vi "RT Driver VI.vi"(7 "Operation":T1, 11 "Device Reference in":T2 format="%.0x") -> (0 "Error Code":i32)   [LabVIEW 2020, in "FPGA Addon Engine.lvlib"]
uses:
  FPGA Addon Engine.lvlib
  <vilib>/rvi/interface/nirviCloseFPGA/nirviCloseFPGA.xnode
  <vilib>/NI VeriStand/Custom Device API/Custom Device API.lvlib
  Processes/Input DMA Engine.vi
  <vilib>/rvi/interface/nirviMethod/nirviMethod.xnode
  Processes/Output DMA Engine.vi
  <vilib>/NI/NIVS Inline Async API/_VS Inline Async API/VS Inline Async API/VS Inline Async API.lvclass
  <vilib>/NI/NIVS Inline Async API/_VS Inline Async API/VS Inline Async API/Types/Error Handling Settings.ctl
  <vilib>/rvi/interface/nirviMethod/StockFPGA_InlinedMethodWaitForSingleIRQ.vi
  <vilib>/FPGAPlugInAG/Dynamic/niLvFpga_WaitOnIrq_Dynamic.vi
  <vilib>/FPGAPlugInAG/Dynamic/niLvFpga_AcknowledgeIrq_Dynamic.vi
  <vilib>/FPGAPlugInAG/Dynamic/niLvFpga_Close_Dynamic.vi
  <vilib>/NI VeriStand/Custom Device Waveform API/Multiple Waveforms Write (DBL)/Multiple Waveforms Write (DBL).lvclass
  <vilib>/NI VeriStand/Custom Device Waveform API/Single Waveform Read (DBL)/Single Waveform Read (DBL).lvclass
  <vilib>/NI VeriStand/Custom Device API/Custom Device Item Ref.ctl
  <vilib>/NI VeriStand/Custom Device API/Hardware Interface Driver VI Operation.ctl
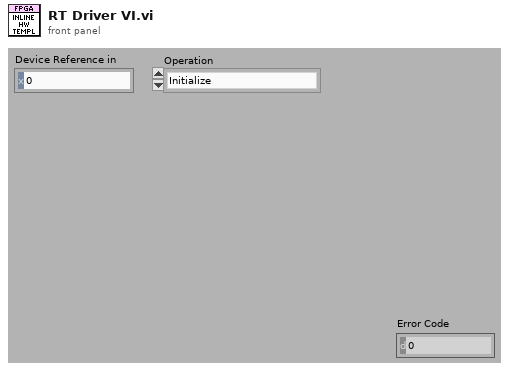
[diagram p1: front panel]
types:
  T1 = typedef "Custom Device API.lvlib/Hardware Interface Driver VI Operation.ctl" = enum16{"Initialize", "Start", "Read Data from HW", "Write Data to HW", "Close"}
  T2 = typedef "Custom Device API.lvlib/Custom Device Item Ref.ctl" = u64
  T3 = typedef "FPGA Addon Engine.lvlib/State Variables.ctl" = cluster{"FPGA Ref":refnum<k20>, "IncomingRegisters.Refs":T4[], "IncomingDMA.Refs":T7[], "OutgoingRegisters.Refs":T4[], "OutgoingDMA.Refs":T12[], "Compiled":T14}
  T4 = typedef "FPGA Addon Engine.lvlib/Register Settings.ctl" = cluster{"Name":string, "Data Type":T5, "session":u32, "Scalar Type":T6, "Index":i32, "Length":i32, "attributes":variant, "default value":variant, "RegisterOffset":u32}
  T5 = typedef "FPGA Addon Shared.lvlib/FPGA Addon Data Type.ctl" = enum8{"<Null>", "I8", "I16", "I32", "I64", "U8", "U16", "U32", "U64", "SGL", "Boolean", "Analog PWM In Settings", "Analog PWM In", "Digital PWM In Settings", "Digital PWM In", "Digital PWM Out", "Sine Out", "FXP", "FXP+/-24.5", "FXP+/-16.5", "FXP+/-32.8", "FXP+/-64.32", "FXP+/-16.7", "FXP+/-20.5", "FXP+/-27.5", "FXP+/-32.16", "FXP+16.3", "FXP+18.3", "Digital Static In", "Digital Static Out", "Digital Static In Settings", "Digital WSS Out", "Quad Encoder Settings", "Quad Encoder In", "Group"}
  T6 = typedef "FPGA Addon Shared.lvlib/Scalar Type.ctl" = enum16{"Standard", "Bitpacked"}
  T7 = typedef "FPGA Addon Engine.lvlib/DMA Input References.ctl" = cluster{"Addon Name":string, "Waveform Ref":refnum<class "Multiple Waveforms Write (DBL).lvclass">, "DMA Name":string, "DMA Settings":T8, "Refs":T11}
  T8 = typedef "FPGA Addon Shared.lvlib/DMA Settings.ctl" = cluster{"Number of Channels":u8, "Delacing Scheme":T9, "Update Rate":u32, "dt":dbl, "Mode":T10, "Number of Samples":u32, "DMA Host Buffer":u32}
  T9 = typedef "FPGA Addon Shared.lvlib/Delacing Scheme.ctl" = enum8{"Interleaved", "Bitpacked"}
  T10 = typedef "FPGA Addon Shared.lvlib/DMA Acquisition Mode.ctl" = enum8{"Continuous", "Triggered Finite"}
  T11 = typedef "FPGA Addon Engine.lvlib/DMA Input Refs.ctl" = cluster{"Data Type":T5, "DMA_SGL":refnum<k20>, "DMA_U64":refnum<k20>, "DMA_I64":refnum<k20>, "DMA_FXP+/-32.8":refnum<k20>, "DMA_FXP+/-64.32":refnum<k20>, "DMA_U32":refnum<k20>, "DMA_U16":refnum<k20>, "DMA_U8":refnum<k20>, "DMA_I32":refnum<k20>, "DMA_I16":refnum<k20>, "DMA_I8":refnum<k20>, "DMA_FXP+/-32.16":refnum<k20>}
  T12 = typedef "FPGA Addon Engine.lvlib/DMA Output References.ctl" = cluster{"Addon Name":string, "Waveforms":refnum<class "Single Waveform Read (DBL).lvclass">[], "DMA Name":string, "Refs":T13}
  T13 = typedef "FPGA Addon Engine.lvlib/DMA Output Refs.ctl" = cluster{"Data Type":T5, "DMA_SGL":refnum<k20>, "DMA_U64":refnum<k20>, "DMA_I64":refnum<k20>, "DMA_FXP+/-32.8":refnum<k20>, "DMA_FXP+/-64.32":refnum<k20>, "DMA_U32":refnum<k20>, "DMA_U16":refnum<k20>, "DMA_U8":refnum<k20>, "DMA_I32":refnum<k20>, "DMA_I16":refnum<k20>, "DMA_I8":refnum<k20>, "DMA_FXP+/-32.16":refnum<k20>}
  T14 = typedef "FPGA Addon Shared.lvlib/Compiled.Settings.ctl" = cluster{"Name":string, "IncomingRegisters.Settings":T15[], "IncomingRegisters.Refs":cluster{"Refs":T17[], "Values":dbl[]}, "OutgoingRegisters.Settings":T15[], "OutgoingRegisters.Refs":cluster{"Refs":T17[], "Values":dbl[]}, "Incoming.Size":i32, "Outgoing.Size":i32, "IncomingDMA.Settings":T19[], "OutgoingDMA.Settings":T19[], "FPGA.Settings":T21, "Target.Type":T22}
  T15 = typedef "FPGA Addon Shared.lvlib/Compiled.RegisterSettings.ctl" = cluster{"Scalar Type":T6, "Index":i32, "Length":i32, "Register":T16}
  T16 = typedef "FPGA Addon Shared.lvlib/Register Information.ctl" = cluster{"Name":string, "Data Type":T5, "Default Value":variant, "Attributes":variant}
  T17 = typedef "Custom Device API.lvlib/Block Data Reference.ctl" = cluster{"Data Reference":T18, "Offset":u64, "Length":u64}
  T18 = typedef "Custom Device API.lvlib/Data Reference.ctl" = i32
  T19 = typedef "FPGA Addon Shared.lvlib/Compiled.DMASettings.ctl" = cluster{"Name":string, "Data Type":T5, "DMA.Settings":T8, "DMA.VSRefs":T20[]}
  T20 = typedef "Custom Device API.lvlib/Waveform Data Reference.ctl" = i32
  T21 = typedef "FPGA Addon Shared.lvlib/FPGA Settings.ctl" = cluster{"Bitfile path":path, "RIO Device Address":string, "Group":bool}
  T22 = typedef "Custom Device API.lvlib/Custom Device Target Type.ctl" = enum16{"PharLap", "VxWorks", "Windows", "Linux_32_ARM", "Linux_x64"}
  T23 = cluster{"Vars":T3, "Async?":bool, "Async":refnum<class "VS Inline Async API.lvclass">}
  T24 = typedef "VS Inline Async API.lvlib/VS Inline Async API.lvclass/Error Handling Settings.ctl" = cluster{"Write to SystemLog (F)":bool}
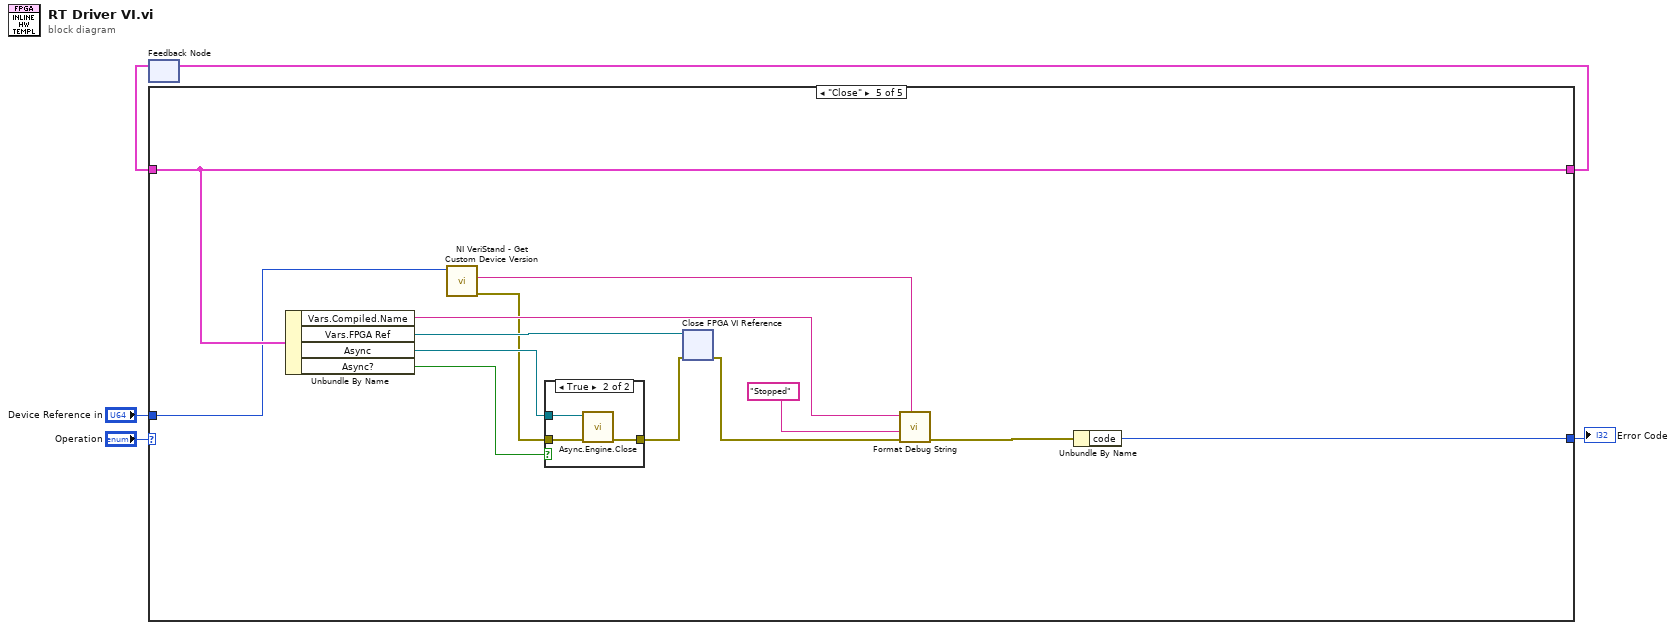
[diagram p0: block diagram]
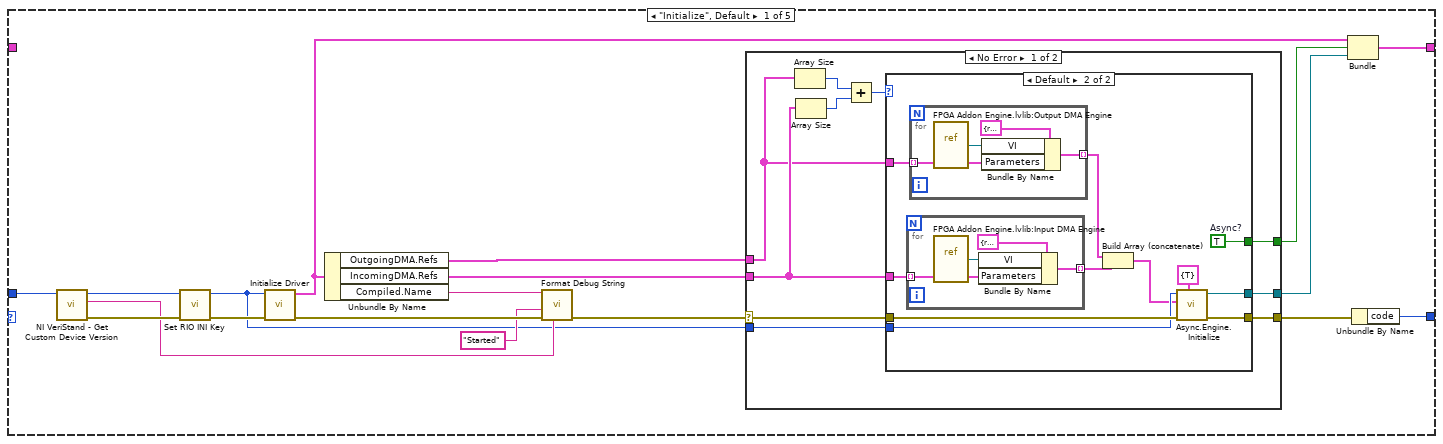
[diagram p2: hidden frame]
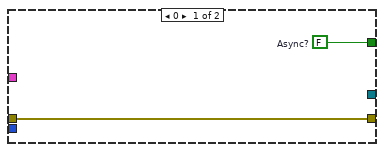
[diagram p3: hidden frame]
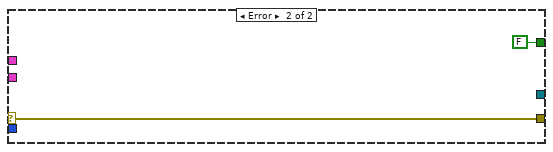
[diagram p4: hidden frame]
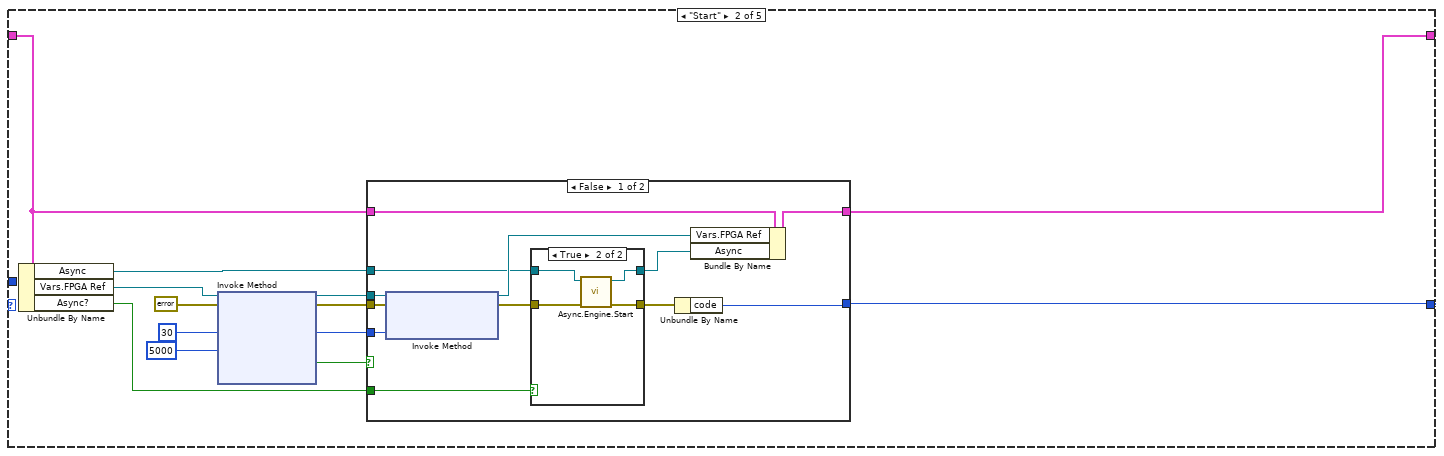
[diagram p5: hidden frame]
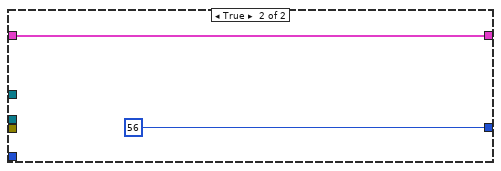
[diagram p7: hidden frame]
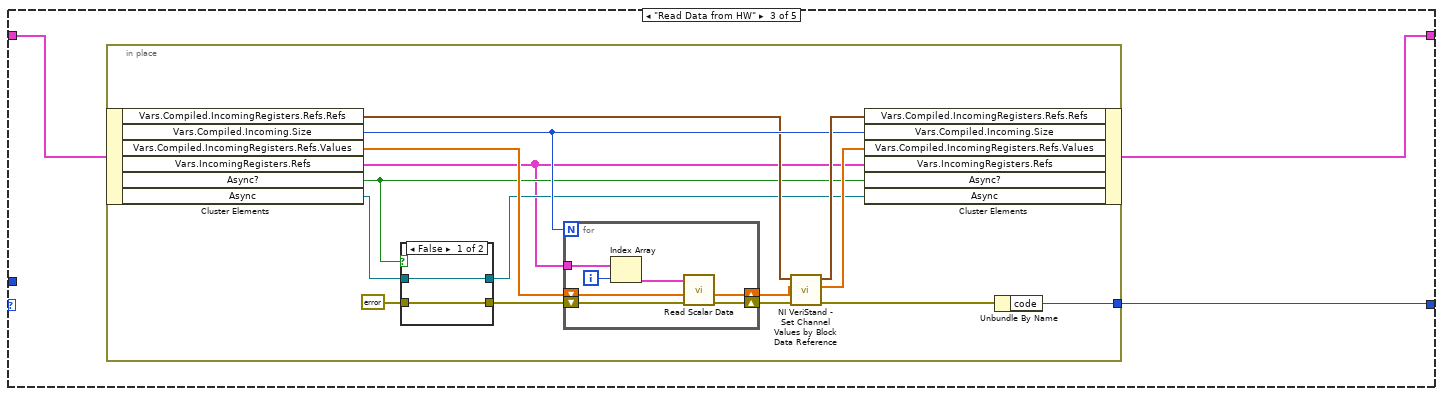
[diagram p8: hidden frame]
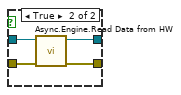
[diagram p9: hidden frame]
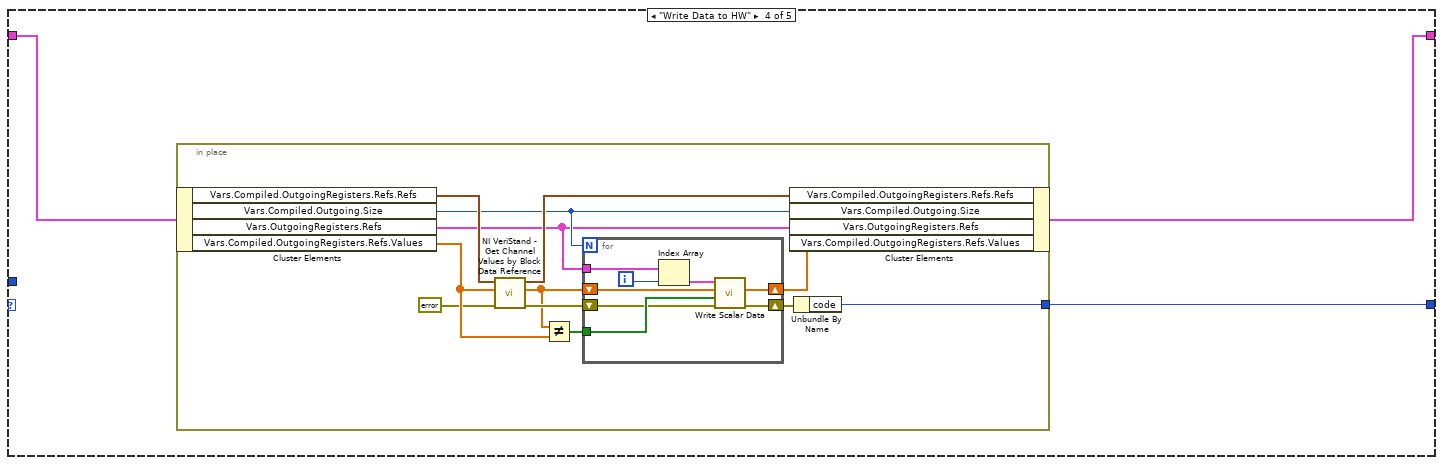
[diagram p10: hidden frame]
diagram:
  n1 = feedback #1() -> (w3:T23)  [unwired: 1 out]
  n2 = case shown="\"Close\"" "Operation" {
    tunnel: [w23 w66 w91 w121 w154] -> w4
    tunnel: w3 -> [_ w67 w89 w122 w154]
    tunnel: "Device Reference in" -> [w13 _ _ _ w149]
    tunnel: [w22 w68 w90 w120 w155] -> w1
    frame "Initialize", Default {
      n3 = call <vilib>:"NI VeriStand - Get Custom Device Version.vi"("Device Ref in"=w13) -> ("error out"=w14:errorcluster, "Value"=w11:string, "Device Ref out"=w7:T2)  [unwired: 8 in]
      n4 = call "Set RIO INI Key.vi"("error in (no error)"=w14, "Section Ref in"=w7) -> ("error out"=w21:errorcluster, "Section Ref out"=w6:T2)  [unwired: 8 in]
      n5 = call "Initialize Driver.vi"("error in (no error)"=w21, "Section Ref in"=w6) -> ("error out"=w12:errorcluster, "Vars"=w15:T3)  [unwired: 8 in]
      n6 = Unbundle By Name(w15) -> ("OutgoingDMA.Refs"=w17:T12[], "IncomingDMA.Refs"=w18:T7[], "Compiled.Name"=w10:string)
      n7 = call "Format Debug String.vi"("Version"=w11, "error in (no error)"=w12, "State"="Started" ("string"), "Name"=w10) -> ("error out"=w8:errorcluster)  [unwired: 7 in]
      n8 = case shown="No Error" w8 {
        selector: w8 -> [w24 w56]
        tunnel: [w33 w56] -> w20
        tunnel: [w32 _] -> w19
        tunnel: w18 -> [w31 _]
        tunnel: w17 -> [w30 _]
        tunnel: [w26 FALSE ("Async?")] -> w16
        tunnel: w6 -> [w25 _]
        frame No Error {
          n9 = Array Size(array=w30) -> (size(s)=w29:i32)
          n10 = Array Size(array=w31) -> (size(s)=w28:i32)
          n11 = Add(x=w29, y=w28) -> (x+y=w27:i32)
          n12 = case shown="Default" w27 {
            tunnel: w24 -> [w35 w43]
            tunnel: [w35 w42] -> w33
            tunnel: [_ w41] -> w32
            tunnel: w31 -> [_ w39]
            tunnel: w30 -> [_ w46]
            tunnel: [w34 w44] -> w26
            tunnel: w25 -> [_ w40]
            frame 0 {
              w34 = FALSE  # Async?
            }
            frame Default {
              w44 = TRUE  # Async?
              n13 = for {
                tunnel: w39 -> [w47] mode=indexing
                tunnel: [w49] -> w38 mode=indexing
                n14 = vi-ref "FPGA Addon Engine.lvlib:Input DMA Engine.vi"() -> (w48:refnum<vi>)
                n15 = Bundle By Name(cluster=cluster{"VI":refnum<vi>, "Parameters":variant} {"VI"=refnum, "Parameters"=variant} ("Process"), "VI"=w48, "Parameters"=w47) -> (w49:cluster{"VI":refnum<vi>, "Parameters":variant})
              }
              n16 = for {
                tunnel: w46 -> [w53] mode=indexing
                tunnel: [w52] -> w45 mode=indexing
                n17 = vi-ref "FPGA Addon Engine.lvlib:Output DMA Engine.vi"() -> (w51:refnum<vi>)
                n18 = Bundle By Name(cluster=cluster{"VI":refnum<vi>, "Parameters":variant} {"VI"=refnum, "Parameters"=variant} ("Process"), "VI"=w51, "Parameters"=w53) -> (w52:cluster{"VI":refnum<vi>, "Parameters":variant})
              }
              n19 = Build Array (concatenate)(w45, w38) -> (w37:cluster{"VI":refnum<vi>, "Parameters":variant}[])
              n20 = call <vilib>:"Async.Engine.Initialize.vi"("Error Log Settings"=T24 {"Write to SystemLog (F)"=TRUE}, "error in (no error)"=w43, "Processes"=w37, "Custom Device Ref"=w40) -> ("error out"=w42:errorcluster, "Async"=w41:refnum<class "VS Inline Async API.lvclass">)  [unwired: 6 in]
            }
          }
        }
        frame Error {
        }
      }
      n21 = Bundle("Vars"=w15, "Async?"=w16, "Async"=w19) -> (w23:T23)  [unwired: 1 out]
      n22 = Unbundle By Name(w20) -> ("code"=w22:i32)
    }
    frame "Start" {
      w62 = 30 ("IRQ Number(s)")
      n23 = Unbundle By Name(w67) -> ("Async"=w58:refnum<class "VS Inline Async API.lvclass">, "Vars.FPGA Ref"=w65:refnum<k20>, "Async?"=w60:bool)
      n24 = xnode "Invoke Method"("FPGA VI Reference In"=w65, "error in"=errorcluster {"status"=FALSE, "code"=0, "source"=""}, "IRQ Number(s)"=w62, "Timeout (ms)"=5000) -> ("FPGA VI Reference Out"=w64:refnum<k20>, "error out"=w63:errorcluster, "Timed Out"=w59:bool)  [unwired: 1 out]
      n25 = case shown="False" w59 {
        tunnel: [w80 56 ("code")] -> w68
        tunnel: w67 -> [w79 w88]
        tunnel: [w78 w88] -> w66
        tunnel: w64 -> [w77 _]
        tunnel: w63 -> [w76 _]
        tunnel: w62 -> [w75 _]
        tunnel: w60 -> [w72 _]
        tunnel: w58 -> [w71 _]
        frame False {
          n26 = xnode "Invoke Method"("FPGA VI Reference In"=w77, "error in"=w76, "IRQ Number(s)"=w75) -> ("FPGA VI Reference Out"=w74:refnum<k20>, "error out"=w69:errorcluster)
          n27 = case shown="True" w72 {
            tunnel: w69 -> [w82 w86]
            tunnel: [w82 w85] -> w73
            tunnel: w71 -> [w81 w84]
            tunnel: [w81 w83] -> w70
            frame False {
            }
            frame True {
              n28 = call <vilib>:"Async.Engine.Start.vi"("error in (no error)"=w86, "VS Inline Async API in"=w84) -> ("error out"=w85:errorcluster, "VS Inline Async API out"=w83:refnum<class "VS Inline Async API.lvclass">)  [unwired: 8 in]
            }
          }
          n29 = Unbundle By Name(w73) -> ("code"=w80:i32)
          n30 = Bundle By Name(cluster=w79, "Vars.FPGA Ref"=w74, "Async"=w70) -> (w78:T23)
        }
        frame True {
        }
      }
    }
    frame "Read Data from HW" {
      n31 = in-place {
        in-place-border: [w98] -> w90
        n32 = in-place-cluster #2(w89) -> ("Vars.Compiled.IncomingRegisters.Refs.Refs"=w100:T17[], "Vars.Compiled.Incoming.Size"=w102:i32, "Vars.Compiled.IncomingRegisters.Refs.Values"=w106:dbl[], "Vars.IncomingRegisters.Refs"=w92:T4[], "Async?"=w94:bool, "Async"=w96:refnum<class "VS Inline Async API.lvclass">)
        n33 = case shown="False" w94 {
          tunnel: w96 -> [w108 w112]
          tunnel: [w107 w111] -> w97
          tunnel: [w108 w110] -> w95
          tunnel: errorcluster {"status"=FALSE, "code"=0, "source"=""} ("error in") -> [w107 w109]
          frame False {
          }
          frame True {
            n34 = call <vilib>:"Async.Engine.Read Data from HW.vi"("error in"=w109, "Async in"=w112) -> ("error out"=w111:errorcluster, "Async out"=w110:refnum<class "VS Inline Async API.lvclass">)  [unwired: 8 in]
          }
        }
        n35 = for {
          N: w102 -> [_]
          shift-right: [w115] -> w103
          shift-left: w106 -> [w116]
          shift-right: [w118] -> w101
          shift-left: w97 -> [w113]
          tunnel: w92 -> [w119]
          i -> [w117]
          n36 = Index Array(array=w119, index=w117) -> (element=w114:T4)
          n37 = call "Read Scalar Data.vi"("error in (no error)"=w113, "Values"=w116, "Cluster"=w114) -> ("error out"=w118:errorcluster, "Values"=w115:dbl[])  [unwired: 7 in]
        }
        n38 = call <vilib>:"NI VeriStand - Set Channel Values by Block Data Reference.vi"("error in (no error)"=w101, "Values Array in"=w103, "Block Data Ref"=w100) -> ("error out"=w99:errorcluster, "Values Array out"=w104:dbl[], "Block Data Ref dup"=w105:T17[])  [unwired: 6 in]
        n39 = in-place-cluster #2("Vars.Compiled.IncomingRegisters.Refs.Refs"=w105, "Vars.Compiled.Incoming.Size"=w102, "Vars.Compiled.IncomingRegisters.Refs.Values"=w104, "Vars.IncomingRegisters.Refs"=w92, "Async?"=w94, "Async"=w95) -> (w91:T23)
        n40 = Unbundle By Name(w99) -> ("code"=w98:i32)
      }
    }
    frame "Write Data to HW" {
      n41 = in-place {
        in-place-border: [w128] -> w120
        n42 = in-place-cluster #3(w122) -> ("Vars.Compiled.OutgoingRegisters.Refs.Refs"=w134:T17[], "Vars.Compiled.Outgoing.Size"=w130:i32, "Vars.OutgoingRegisters.Refs"=w123:T4[], "Vars.Compiled.OutgoingRegisters.Refs.Values"=w126:dbl[])
        n43 = call <vilib>:"NI VeriStand - Get Channel Values by Block Data Reference.vi"("error in (no error)"=errorcluster {"status"=FALSE, "code"=0, "source"=""} ("error in"), "Values Array in"=w126, "Block Data Ref"=w134) -> ("error out"=w131:errorcluster, "Values Array out"=w127:dbl[], "Block Data Ref dup"=w133:T17[])  [unwired: 6 in]
        n44 = Not Equal?(x=w127, y=w126) -> (x != y?=w125:bool[])
        n45 = for {
          N: w130 -> [_]
          shift-right: [w138] -> w132
          shift-left: w127 -> [w142]
          shift-right: [w139] -> w129
          shift-left: w131 -> [w136]
          tunnel: w125 -> [w137]
          tunnel: w123 -> [w141]
          i -> [w140]
          n46 = Index Array(array=w141, index=w140) -> (element=w135:T4)
          n47 = call "Write Scalar Data.vi"("error in (no error)"=w136, "Changed?"=w137, "Values"=w142, "Cluster"=w135) -> ("error out"=w139:errorcluster, "Values"=w138:dbl[])  [unwired: 6 in]
        }
        n48 = in-place-cluster #3("Vars.Compiled.OutgoingRegisters.Refs.Refs"=w133, "Vars.Compiled.Outgoing.Size"=w130, "Vars.OutgoingRegisters.Refs"=w123, "Vars.Compiled.OutgoingRegisters.Refs.Values"=w132) -> (w121:T23)
        n49 = Unbundle By Name(w129) -> ("code"=w128:i32)
      }
    }
    frame "Close" {
      n50 = Unbundle By Name(w154) -> ("Vars.Compiled.Name"=w144:string, "Vars.FPGA Ref"=w152:refnum<k20>, "Async"=w150:refnum<class "VS Inline Async API.lvclass">, "Async?"=w151:bool)
      n51 = call <vilib>:"NI VeriStand - Get Custom Device Version.vi"("Device Ref in"=w149) -> ("error out"=w143:errorcluster, "Value"=w145:string)  [unwired: 8 in, 1 out]
      n52 = case shown="True" w151 {
        tunnel: [w156 w159] -> w153
        tunnel: w150 -> [_ w158]
        tunnel: w143 -> [w156 w157]
        frame False {
        }
        frame True {
          n53 = call <vilib>:"Async.Engine.Close.vi"("error in (no error)"=w157, "Async in"=w158) -> ("error out"=w159:errorcluster)  [unwired: 8 in, 1 out]
        }
      }
      n54 = xnode "Close FPGA VI Reference"("FPGA VI Reference In"=w152, "error in"=w153) -> ("error out"=w146:errorcluster)
      n55 = call "Format Debug String.vi"("Version"=w145, "error in (no error)"=w146, "State"="Stopped" ("string"), "Name"=w144) -> ("error out"=w147:errorcluster)  [unwired: 7 in]
      n56 = Unbundle By Name(w147) -> ("code"=w155:i32)
    }
  }
  "Error Code" <- w1
  n57 = feedback-in #1(w4) -> ()
